vi "Set Layout.vi"(8 "error in (no error)":errorcluster, 9 "Snap plot":refnum<vi>, 10 "XY Plot":refnum<vi>, 11 "XY Plotter":refnum<class "XY Plotter.lvclass">) -> (0 "error out":errorcluster, 3 "XY Plotter out":refnum<class "XY Plotter.lvclass">)   [LabVIEW 2025, in "XY Plotter.lvlib" / "XY Plotter.lvclass"]
uses:
  XY Plotter.lvclass
  XY Plotter.lvclass/XY Plotter.ctl
  XY Plotter configuration/XY Plotter configuration.lvclass/XY Plotter configuration.ctl
  XY Plotter configuration/Read XY Plotter.vi
  XY Plotter configuration/XY Plotter configuration.lvclass
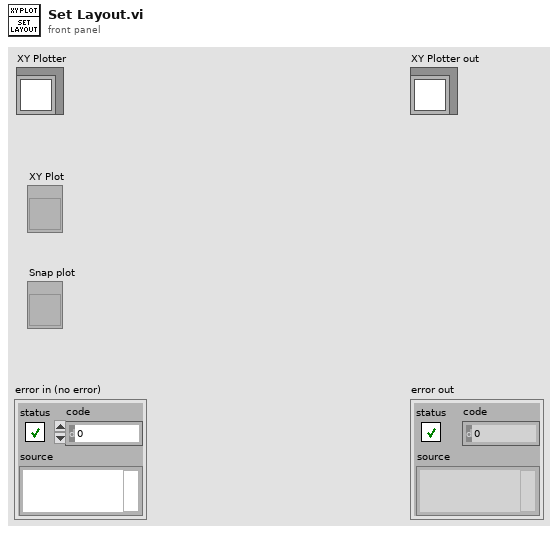
[diagram p1: front panel]
types:
  T1 = typedef "XY Plotter.lvlib/XY Plotter configuration.lvclass/XY Plotter.ctl" = cluster{"Data Rate":i32, "Y-Scales":cluster{"Label":string, "Max":dbl, "Min":dbl, "Unit":enum16{"---", "V", "mA", "sec", "dB", "deg", "in/s", "in", "lbf", "Hz", "psi", "gpm"}, "Visible":bool}[], "Note":string, "History Length":i32, "DataLog Path":path, "Plot type":bool, "X-Scales":cluster{"Label":string, "Max":dbl, "Min":dbl, "Unit":enum16{"---", "V", "mA", "sec", "dB", "deg", "in/s", "in", "lbf", "Hz", "psi", "gpm"}, "Visible":bool}[], "Plot List":cluster{"Plot Name":string, "X Scale Index":u32, "Y Scale Index":u32, "Visible":bool}[]}
  T2 = cluster{"Plot Name":string, "X Scale Index":u32, "Y Scale Index":u32, "Visible":bool}[]
  T3 = cluster{"Label":string, "Max":dbl, "Min":dbl, "Unit":enum16{"---", "V", "mA", "sec", "dB", "deg", "in/s", "in", "lbf", "Hz", "psi", "gpm"}, "Visible":bool}[]
  T4 = enum16{"---", "V", "mA", "sec", "dB", "deg", "in/s", "in", "lbf", "Hz", "psi", "gpm"}
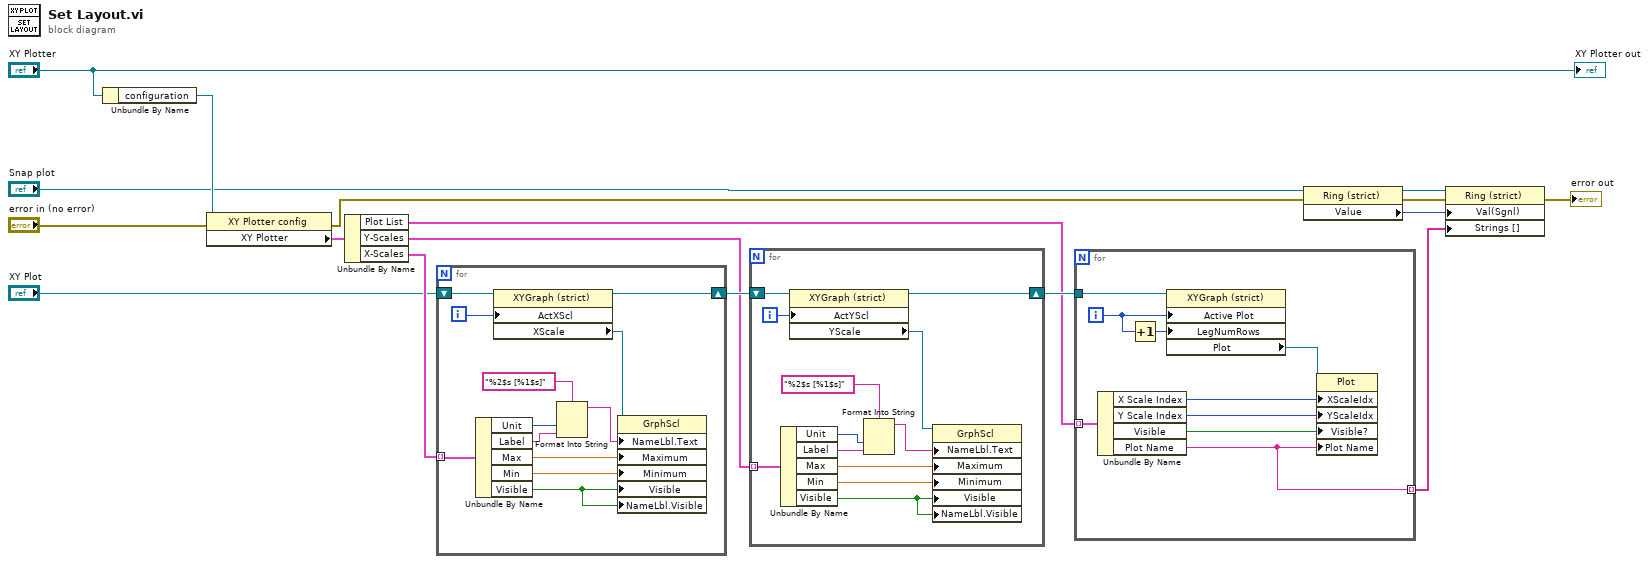
[diagram p0: block diagram]
diagram:
  n1 = Unbundle By Name("XY Plotter") -> ("configuration"=w4:refnum<class "XY Plotter configuration.lvclass">)
  n2 = property class="XY Plotter config"(reference=w4, error in="error in (no error)") -> (error out=w7:errorcluster, "XY Plotter"=w14:T1)  [unwired: 1 out]
  n3 = Unbundle By Name(w14) -> ("Plot List"=w11:T2, "Y-Scales"=w12:T3, "X-Scales"=w13:T3)
  n4 = for {
    tunnel: w13 -> [w20] mode=indexing
    shift-right: [w21] -> w15
    shift-left: "XY Plot" -> [w19]
    i -> [w18]
    n5 = Unbundle By Name(w20) -> ("Unit"=w23:T4, "Label"=w25:string, "Max"=w27:dbl, "Min"=w28:dbl, "Visible"=w29:bool)
    n6 = property class="XYGraph (strict)"(reference=w19, "ActXScl"=w18) -> (reference out=w21:refnum<vi>, "XScale"=w22:refnum<vi>)  [unwired: 1 in, 1 out]
    n7 = Format Into String(format string="%2$s [%1$s]" ("Name Label.Text"), w23, w25) -> (resulting string=w26:string)  [unwired: 2 in, 1 out]
    n8 = property class="GrphScl"(reference=w22, "NameLbl.Text"=w26, "Maximum"=w27, "Minimum"=w28, "Visible"=w29, "NameLbl.Visible"=w29) -> ()  [unwired: 1 in, 2 out]
  }
  n9 = for {
    tunnel: w12 -> [w39] mode=indexing
    shift-right: [w35] -> w16
    shift-left: w15 -> [w41]
    i -> [w40]
    n10 = Unbundle By Name(w39) -> ("Unit"=w33:T4, "Label"=w32:string, "Max"=w37:dbl, "Min"=w36:dbl, "Visible"=w30:bool)
    n11 = property class="XYGraph (strict)"(reference=w41, "ActYScl"=w40) -> (reference out=w35:refnum<vi>, "YScale"=w38:refnum<vi>)  [unwired: 1 in, 1 out]
    n12 = Format Into String(format string="%2$s [%1$s]" ("Name Label.Text"), w33, w32) -> (resulting string=w31:string)  [unwired: 2 in, 1 out]
    n13 = property class="GrphScl"(reference=w38, "NameLbl.Text"=w31, "Maximum"=w37, "Minimum"=w36, "Visible"=w30, "NameLbl.Visible"=w30) -> ()  [unwired: 1 in, 2 out]
  }
  n14 = for {
    tunnel: w11 -> [w46] mode=indexing
    tunnel: [w44] -> w17 mode=indexing
    tunnel: w16 -> [w48]
    i -> [w47]
    n15 = Unbundle By Name(w46) -> ("X Scale Index"=w42:u32, "Y Scale Index"=w43:u32, "Visible"=w45:bool, "Plot Name"=w44:string)
    n16 = Increment(x=w47) -> (x+1=w49:i32)
    n17 = property class="XYGraph (strict)"(reference=w48, "Active Plot"=w47, "LegNumRows"=w49) -> ("Plot"=w50:refnum<vi>)  [unwired: 1 in, 2 out]
    n18 = property class="Plot"(reference=w50, "XScaleIdx"=w42, "YScaleIdx"=w43, "Visible?"=w45, "Plot Name"=w44) -> ()  [unwired: 1 in, 2 out]
  }
  n19 = property class="Ring (strict)"(reference="Snap plot", error in=w7) -> (reference out=w10:refnum<vi>, error out=w8:errorcluster, "Value"=w9:u16)
  n20 = property class="Ring (strict)"(reference=w10, error in=w8, "Val(Sgnl)"=w9, "Strings []"=w17) -> (error out=→"error out":errorcluster)  [unwired: 1 out]
  "XY Plotter out" <- "XY Plotter"
